vi "query_simple.vi"(8 "error in (no error)":errorcluster, 11 "VISA resource name":refnum<visa-resource-name>) -> (0 "error out":errorcluster, 2 "Reply":string)   [LabVIEW 2026]
panel:
  in  "stop":bool
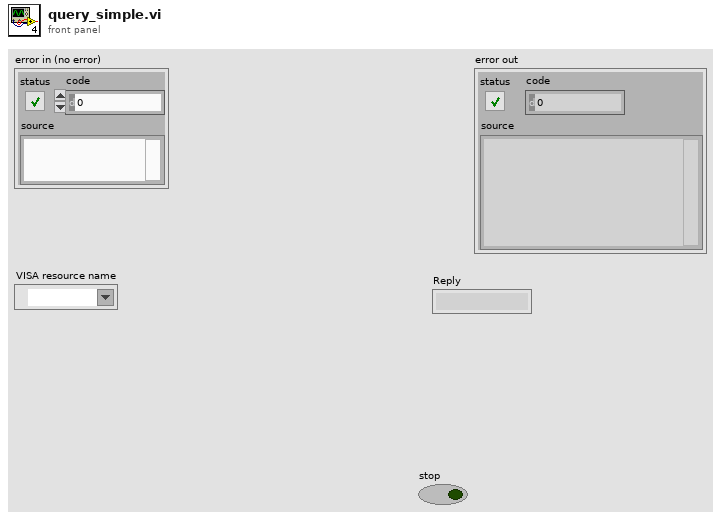
[diagram p1: front panel]
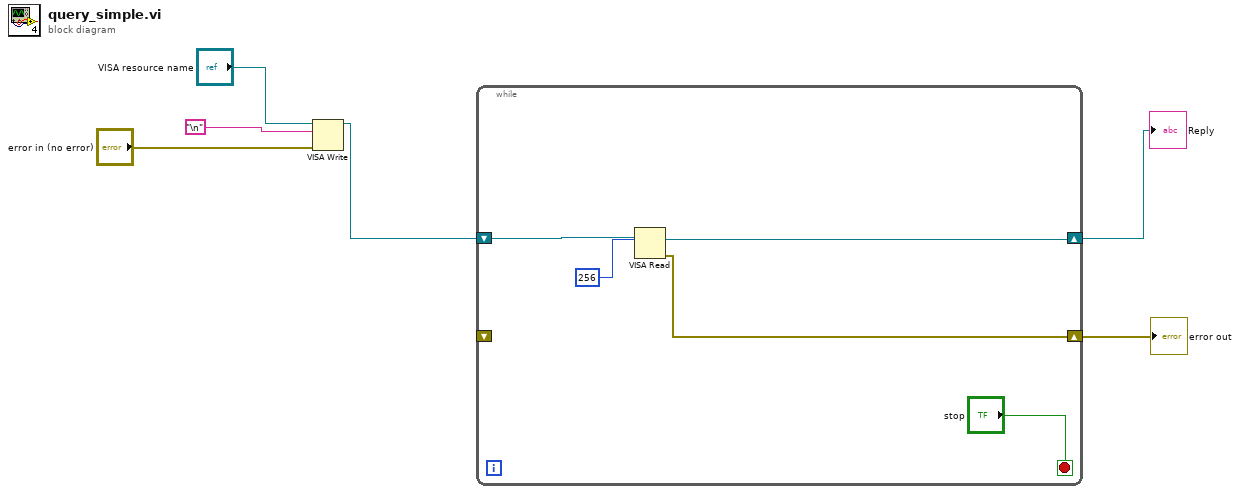
[diagram p0: block diagram]
diagram:
  n1 = VISA Write(VISA resource name="VISA resource name", write buffer="\n", error in (no error)="error in (no error)") -> (VISA resource name out=w5:refnum<visa-resource-name>)  [unwired: 2 out]
  n2 = while {
    shift-right: [w10] -> w3
    shift-left: w5 -> [w11]
    shift-right: [w7] -> w1
    shift-left: _ -> [_]
    stop <- "stop" stop-if-true
    n3 = VISA Read(VISA resource name=w11, byte count=u32 256) -> (VISA resource name out=w10:refnum<visa-resource-name>, error out=w7:errorcluster)  [unwired: 1 in, 2 out]
  }
  "error out" <- w1
  "Reply" <- w3
